vi "GeneratorUI-Advanced.vi"(8 "error in":errorcluster, 9 "Unattended Mode":bool, 10 "File configurations":T1(array[cluster]), 11 "Top level output path":path) -> (0 "error out":errorcluster)   [LabVIEW 2017]
uses:
  PathConfiguration.vi
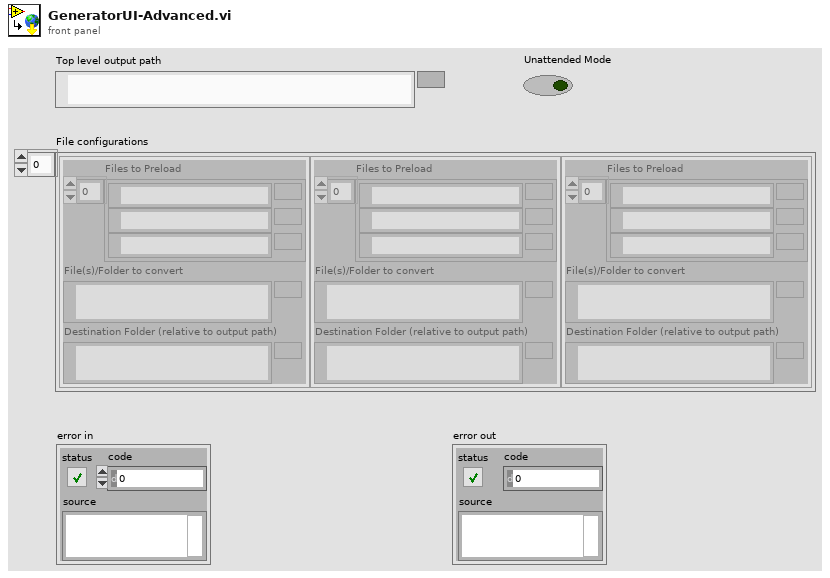
[diagram p1: front panel]
types:
  T1 = cluster{"Files to Preload":path[], "File(s)/Folder to convert":path, "Destination Folder (relative to output path)":path}[]
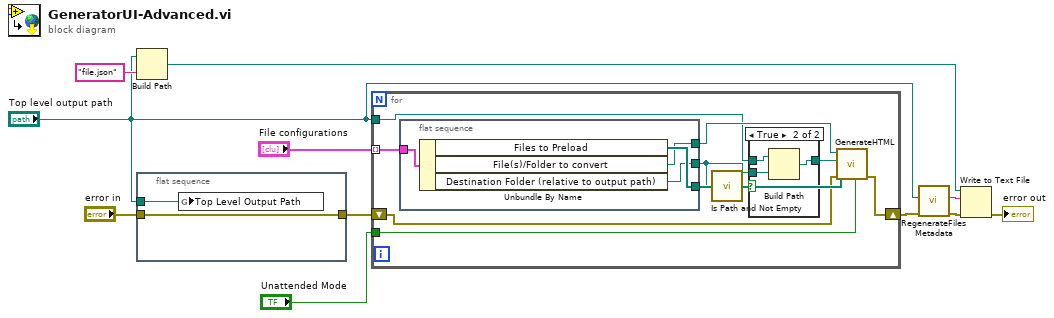
[diagram p0: block diagram]
diagram:
  n1 = Build Path(base path="Top level output path", name or relative path="file.json") -> (appended path=w1:path)
  n2 = flat-sequence {
    tunnel: "Top level output path" -> [w13]
    tunnel: "error in" -> [w12]
    tunnel: [w12] -> w2
    frame #0 {
      n3 = global write "PathConfiguration.vi" "Top Level Output Path"(w13) -> ()
    }
  }
  n4 = for {
    tunnel: "File configurations" -> [w23] mode=indexing
    shift-right: [w19] -> w9
    shift-left: w2 -> [w20]
    tunnel: "Top level output path" -> [w16]
    tunnel: "Unattended Mode" -> [w18]
    n5 = flat-sequence {
      tunnel: w23 -> [w31]
      tunnel: [w30] -> w22
      tunnel: [w29] -> w21
      tunnel: [w28] -> w15
      frame #0 {
        n6 = Unbundle By Name(w31) -> ("Files to Preload"=w30:path[], "File(s)/Folder to convert"=w29:path, "Destination Folder (relative to output path)"=w28:path)
      }
    }
    n7 = call <vilib>:"Is Path and Not Empty.vi"("path"=w15) -> ("Is Path and Not Empty?"=w17:bool)  [unwired: 4 in]
    n8 = case shown="True" w17 {
      tunnel: w16 -> [w24 w27]
      tunnel: w15 -> [_ w26]
      tunnel: [w24 w25] -> w14
      frame False {
      }
      frame True {
        n9 = Build Path(base path=w27, name or relative path=w26) -> (appended path=w25:path)
      }
    }
    n10 = call "GenerateHTML.vi"("Unattended Mode"=w18, "error in (no error)"=w20, "Files to preload"=w22, "Destination Directory"=w14, "Source directory/files"=w21) -> ("error out"=w19:errorcluster)  [unwired: 5 in, 1 out]
  }
  n11 = call "RegenerateFilesMetadata.vi"("error in (no error)"=w9, "Path"="Top level output path") -> ("error out"=w7:errorcluster, "String"=w8:string)  [unwired: 7 in, 1 out]
  n12 = Write to Text File(file (use dialog)=w1, text=w8, error in=w7) -> (error out=→"error out":errorcluster)  [unwired: 1 in, 2 out]
